vi "Execute Tests.vi"(8 "error in (no error)":errorcluster, 10 "Tests":string[](array[string]), 11 "Execution UI In":refnum<class "Execution UI.lvclass">) -> (0 "error out":errorcluster, 3 "Execution UI Out":refnum<class "Execution UI.lvclass">)   [LabVIEW 2020, in "Execution UI.lvclass"]
uses:
  Execution UI.lvclass
  TypeDefs/Execution State.ctl
  Result Model/Result Model.lvclass
  LUnit Test Suite.lvclass
  Framework/Test Runner/Test Runner.lvclass
  Framework/Plugin/Plugin.lvclass
  C:/git/astemes-lunit/source/Runnable.lvclass
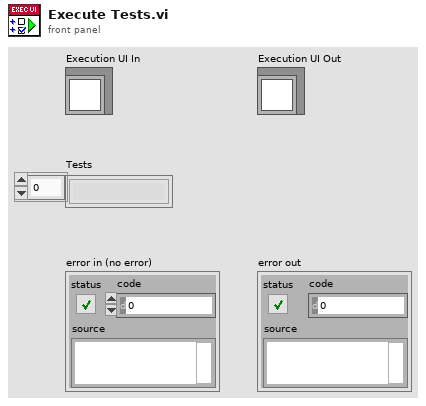
[diagram p1: front panel]
types:
  T1 = typedef "Execution UI.lvclass/Execution State.ctl" = enum16{"Idle", "Running"}
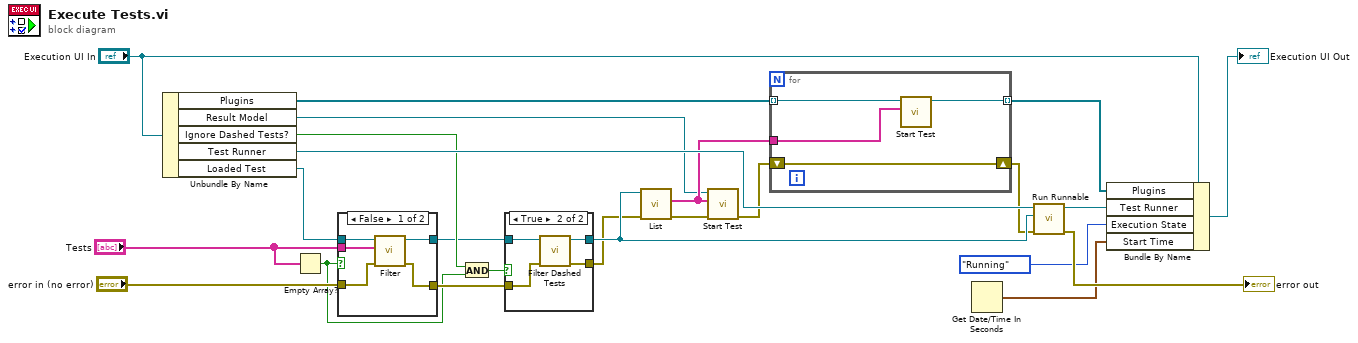
[diagram p0: block diagram]
diagram:
  n1 = Unbundle By Name("Execution UI In") -> ("Plugins"=w8:refnum<class "Plugin.lvclass">[], "Result Model"=w9:refnum<class "Result Model.lvclass">, "Ignore Dashed Tests?"=w17:bool, "Test Runner"=w24:refnum<class "Test Runner.lvclass">, "Loaded Test"=w15:refnum<class "LUnit Test Suite.lvclass">)
  n2 = Empty Array?(array="Tests") -> (empty?=w11:bool)
  n3 = case shown="False" w11 {
    tunnel: "error in (no error)" -> [w29 w31]
    tunnel: w15 -> [w28 w30]
    tunnel: [w27 w30] -> w14
    tunnel: "Tests" -> [w26 _]
    tunnel: [w25 w31] -> w12
    frame False {
      n4 = call "Filter.vi"("error in (no error)"=w29, "Selected Runnables"=w26, "LUnit Test Suite In"=w28) -> ("error out"=w25:errorcluster, "LUnit Test Suite Out"=w27:refnum<class "LUnit Test Suite.lvclass">)  [unwired: 7 in]
    }
    frame True {
    }
  }
  n5 = And(x=w17, y=w11) -> (x .and. y?=w16:bool)
  n6 = case shown="True" w16 {
    tunnel: w12 -> [w32 w34]
    tunnel: [w32 w35] -> w7
    tunnel: w14 -> [w33 w36]
    tunnel: [w33 w37] -> w18
    frame False {
    }
    frame True {
      n7 = call "Filter Dashed Tests.vi"("error in (no error)"=w34, "Test Suite"=w36) -> ("error out"=w35:errorcluster, "Filtered Test Suite"=w37:refnum<class "LUnit Test Suite.lvclass">)  [unwired: 8 in]
    }
  }
  n8 = call "List.vi"("error in (no error)"=w7, "LUnit Test Suite In"=w18) -> ("error out"=w21:errorcluster, "List of Runnables"=w20:string[])  [unwired: 8 in]
  n9 = call "Start Test.vi"("error in (no error)"=w21, "Tests"=w20, "Result Model by Reference In"=w9) -> ("error out"=w3:errorcluster)  [unwired: 8 in]
  n10 = for {
    tunnel: w20 -> [w41]
    tunnel: w8 -> [w39] mode=indexing
    shift-right: [w40] -> w2
    shift-left: w3 -> [w40]
    tunnel: [w38] -> w1 mode=indexing
    n11 = call-dynamic "Start Test.vi"("Tests"=w41, "Plugin in"=w39) -> ("Plugin out"=w38:refnum<class "Plugin.lvclass">)  [unwired: 8 in, 1 out]
  }
  n12 = Get Date/Time In Seconds() -> (seconds since 1Jan1904=w4:timestamp)
  n13 = call-dynamic "Run Runnable.vi"("error in (no error)"=w2, "Runnable"=w18, "Test Runner In"=w24) -> ("error out"=→"error out":errorcluster, "Test Runner Out"=w23:refnum<class "Test Runner.lvclass">)  [unwired: 7 in]
  n14 = Bundle By Name(cluster="Execution UI In", "Plugins"=w1, "Test Runner"=w23, "Execution State"=Execution_State."Running", "Start Time"=w4) -> (→"Execution UI Out":refnum<class "Execution UI.lvclass">)
